vi "C_HDLC_Encode.vi"(8 "error in (no error)":errorcluster, 11 "payload":u8[](array[numeric]) format="%.0x") -> (0 "error out":errorcluster, 3 "frame":u8[](array[numeric]) format="%.0x")   [LabVIEW 2021, in "CANsub_C.lvlib"]
doc: "HDLC-encodes one payload for the CANsub: appends the CRC32 (big-endian), escapes 7E and 7D, and adds the 7E flags at both ends. Allocates on every call: tests and setup only."
uses:
  CANsub_C.lvlib
  codec_vis/CANsub_Codec.lvlib
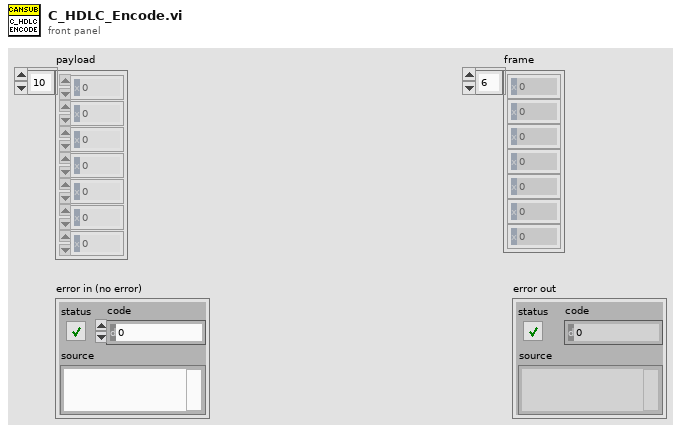
[diagram p1: front panel]
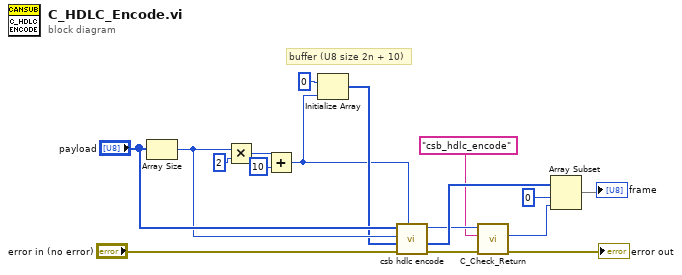
[diagram p0: block diagram]
diagram:
  # "buffer (U8 size 2n + 10)"
  n1 = Array Size(array="payload") -> (size(s)=w12:i32)
  n2 = Multiply(x=w12, y=2) -> (x*y=w14:i32)
  n3 = Add(x=w14, y=10) -> (x+y=w10:i32)
  n4 = Initialize Array(u8 0, w10) -> (w11:u8[])
  n5 = call "csb hdlc encode.vi"("frame_cap"=w10, "error in (no error)"="error in (no error)", "frame"=w11, "len"=w12, "payload"="payload") -> ("error out"=w6:errorcluster, "frame out"=w9:u8[], "function return"=w5:i32)  [unwired: 4 in]
  n6 = call "C_Check_Return.vi"("error in (no error)"=w6, "function name"="csb_hdlc_encode", "function return"=w5) -> ("error out"=→"error out":errorcluster, "length"=w1:i32)  [unwired: 6 in, 1 out]
  n7 = Array Subset(array=w9, index=0, length=w1) -> (→"frame":u8[])
